vi "Unescape INI String.vi"(8 "error in (no error)":errorcluster, 11 "Escaped":string) -> (0 "error out":errorcluster, 3 "Text":string)   [LabVIEW 2024]
doc: "Turns the escapes written by Escape INI String.vi back into characters: a doubled backslash becomes one backslash, backslash-0A a line feed and backslash-0D a carriage return. Used when reading a quoted value from a storage INI file.\n\nGenerated by: Claude"
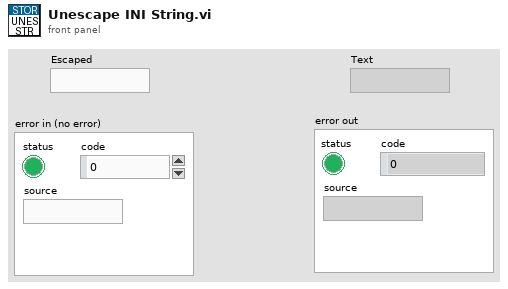
[diagram p1: front panel]
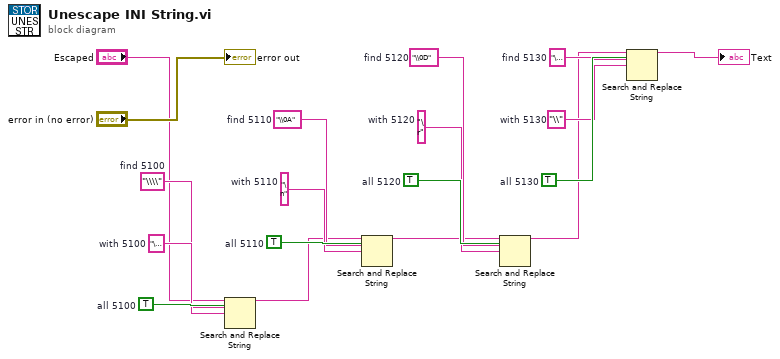
[diagram p0: block diagram]
diagram:
  w17 = TRUE  # all 5130
  w16 = "\\"  # with 5130
  w15 = "\u0001"  # find 5130
  w13 = TRUE  # all 5120
  w12 = "\r"  # with 5120
  w11 = "\\0D"  # find 5120
  w9 = TRUE  # all 5110
  w8 = "\n"  # with 5110
  w7 = "\\0A"  # find 5110
  w5 = TRUE  # all 5100
  w4 = "\u0001"  # with 5100
  w3 = "\\\\"  # find 5100
  n1 = Search and Replace String(replace all?=w5, input string="Escaped", search string=w3, replace string=w4) -> (result string=w6:string)  [unwired: 4 in, 3 out]
  n2 = Search and Replace String(replace all?=w9, input string=w6, search string=w7, replace string=w8) -> (result string=w10:string)  [unwired: 4 in, 3 out]
  n3 = Search and Replace String(replace all?=w13, input string=w10, search string=w11, replace string=w12) -> (result string=w14:string)  [unwired: 4 in, 3 out]
  n4 = Search and Replace String(replace all?=w17, input string=w14, search string=w15, replace string=w16) -> (result string=→"Text":string)  [unwired: 4 in, 3 out]
  "error out" <- "error in (no error)"
